vi "SPARK Configure Closed Loop.vi"   [LabVIEW 2023]
doc: "Configure the closed loop controller of the SPARK."
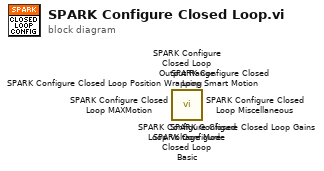
[diagram p0: block diagram]
diagram:
  n1 = call <vilib>:"SPARK Configure Closed Loop Voltage Mode.vi"() -> ()  [unwired: 10 in, 2 out]
  n2 = call <vilib>:"SPARK Configure Closed Loop Smart Motion.vi"() -> ()  [unwired: 10 in, 2 out]
  n3 = call <vilib>:"SPARK Configure Closed Loop MAXMotion.vi"() -> ()  [unwired: 10 in, 2 out]
  n4 = call <vilib>:"SPARK Configure Closed Loop Miscellaneous.vi"() -> ()  [unwired: 10 in, 2 out]
  n5 = call <vilib>:"SPARK Configure Closed Loop Position Wrapping.vi"() -> ()  [unwired: 10 in, 2 out]
  n6 = call <vilib>:"SPARK Configure Closed Loop Output Range.vi"() -> ()  [unwired: 10 in, 2 out]
  n7 = call <vilib>:"SPARK Configure Closed Loop Gains.vi"() -> ()  [unwired: 10 in, 2 out]
  n8 = call <vilib>:"SPARK Configure Closed Loop Basic.vi"() -> ()  [unwired: 10 in, 2 out]
